vi "PSK Demodulator.vi"(0 "PSK Modulated Signal":dbl[](array[numeric]), 1 "Sampling Frequency(Fs)":dbl, 2 "Carrier Frequency (fc)":dbl, 3 "Samples per Bit":i32, 4 "Phase for Binary 1":dbl) -> (5 "Recovered Binary Signal":i32[](array[numeric]))   [LabVIEW 2026]
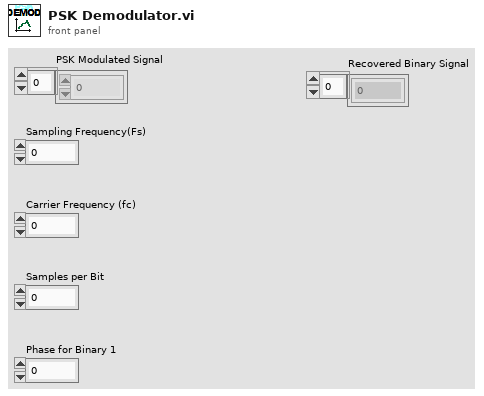
[diagram p1: front panel]
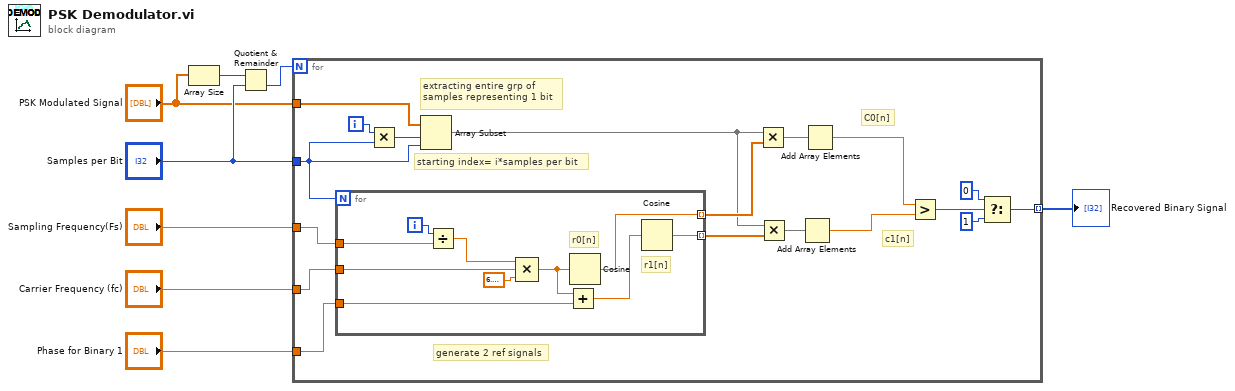
[diagram p0: block diagram]
diagram:
  n1 = Array Size(array="PSK Modulated Signal") -> (size(s)=w8:i32)
  n2 = Quotient & Remainder(x=w8, y="Samples per Bit") -> (floor(x/y)=w7:i32)  [unwired: 1 out]
  n3 = for {
    N: w7 -> [_]
    tunnel: "Samples per Bit" -> [w21]
    tunnel: "PSK Modulated Signal" -> [w25]
    tunnel: "Sampling Frequency(Fs)" -> [w23]
    tunnel: "Carrier Frequency (fc)" -> [w22]
    tunnel: [w10] -> w2 mode=indexing
    tunnel: "Phase for Binary 1" -> [w9]
    i -> [w26]
    # "starting index= i*samples per bit"
    # "extracting entire grp of \nsamples representing 1 bit"
    # "generate 2 ref signals"
    # "c1[n]"
    # "C0[n]"
    n4 = for {
      N: w21 -> [_]
      tunnel: w23 -> [w35]
      tunnel: w22 -> [w33]
      tunnel: [w29] -> w20 mode=indexing
      tunnel: [w28] -> w18 mode=indexing
      tunnel: w9 -> [w27]
      i -> [w36]
      # "r1[n]"
      # "r0[n]"
      n5 = Divide(x=w36, y=w35) -> (x/y=w34:dbl)
      n6 = Compound Arithmetic op=MULTIPLY(w34, w33, 6.283185307179586) -> (w31:dbl)
      n7 = Add(x=w31, y=w27) -> (x+y=w30:dbl)
      n8 = Cosine(x=w31) -> (cos(x)=w29:dbl)
      n9 = Cosine(x=w30) -> (cos(x)=w28:dbl)
    }
    n10 = Multiply(x=w26, y=w21) -> (x*y=w24:i32)
    n11 = Array Subset(array=w25, index=w24, length=w21) -> (w19:dbl[])
    n12 = Multiply(x=w19, y=w20) -> (x*y=w17:dbl[])
    n13 = Multiply(x=w19, y=w18) -> (x*y=w16:dbl[])
    n14 = Add Array Elements(numeric array=w16) -> (sum=w14:dbl)
    n15 = Add Array Elements(numeric array=w17) -> (sum=w15:dbl)
    n16 = Greater?(x=w15, y=w14) -> (0:w13:bool)
    n17 = Select(t=0, s=w13, f=1) -> (s? t:f=w10:i32)
  }
  "Recovered Binary Signal" <- w2
